vi "Write timeout.vi"(8 "error in (no error)":errorcluster, 10 "timeout (2000 ms)":i32=2000, 11 "Test Suite in":refnum<class "Test Suite.lvclass">) -> (0 "error out":errorcluster, 3 "Test Suite out":refnum<class "Test Suite.lvclass">)   [LabVIEW 2013, in "Caraya.lvlib" / "Test Suite.lvclass"]
uses:
  Test Suite.lvclass
  Test Suite.lvclass/Test Suite.ctl
  Properties.Suite/Properties.Suite.lvclass/Properties.Suite.ctl
  Properties.Suite/Properties.Suite.lvclass
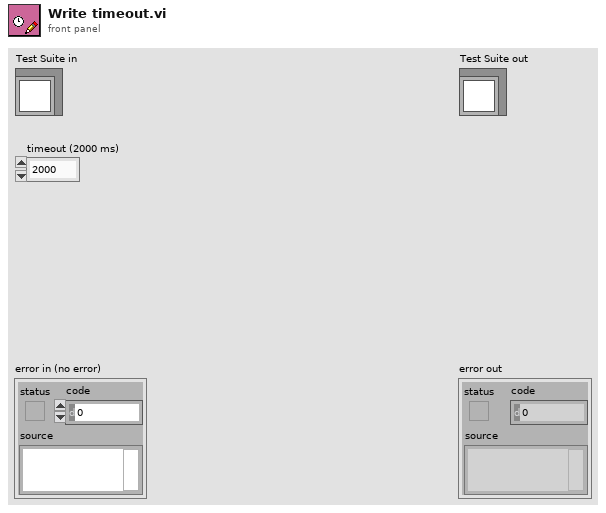
[diagram p1: front panel]
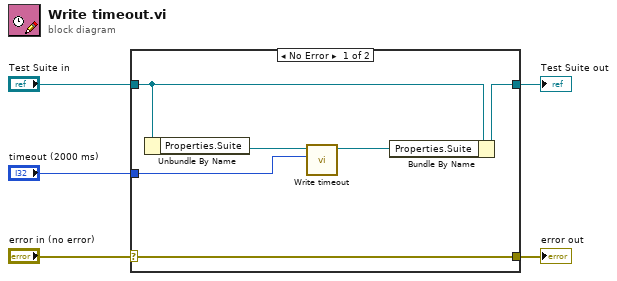
[diagram p0: block diagram]
diagram:
  n1 = case shown="No Error" "error in (no error)" {
    selector: "error in (no error)" -> [w11 w12]
    tunnel: [w11 w12] -> w4
    tunnel: [w10 w13] -> w2
    tunnel: "Test Suite in" -> [w9 w13]
    tunnel: "timeout (2000 ms)" -> [w7 _]
    frame No Error {
      n2 = Unbundle By Name(w9) -> ("Properties.Suite"=w8:refnum<class "Properties.Suite.lvclass">)
      n3 = call "Write timeout.vi"("timeout"=w7, "Properties.Suite in"=w8) -> ("Properties.Suite out"=w6:refnum<class "Properties.Suite.lvclass">)  [unwired: 9 in]
      n4 = Bundle By Name(cluster=w9, "Properties.Suite"=w6) -> (w10:refnum<class "Test Suite.lvclass">)
    }
    frame Error {
    }
  }
  "error out" <- w4
  "Test Suite out" <- w2
